vi "upload.file_multipart_upload.vi"(8 "error in":errorcluster, 10 "File Path":path, 11 "Nominal Client in":refnum<class "Nominal Client.lvclass">) -> (0 "error out":errorcluster, 2 "S3 Path to File":string, 3 "Nominal Client out":refnum<class "Nominal Client.lvclass">)   [LabVIEW 2020, in "Nominal Client.lvclass"]
doc: "Handles the upload of files in a multipart format."
uses:
  Nominal Client.lvclass
  Nominal Client MultiPart Upload/Multipart Upload.lvclass
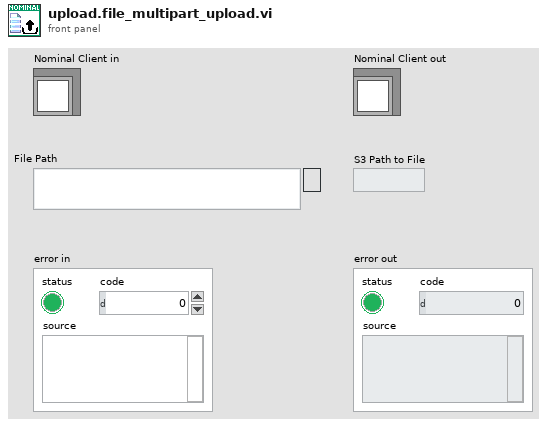
[diagram p1: front panel]
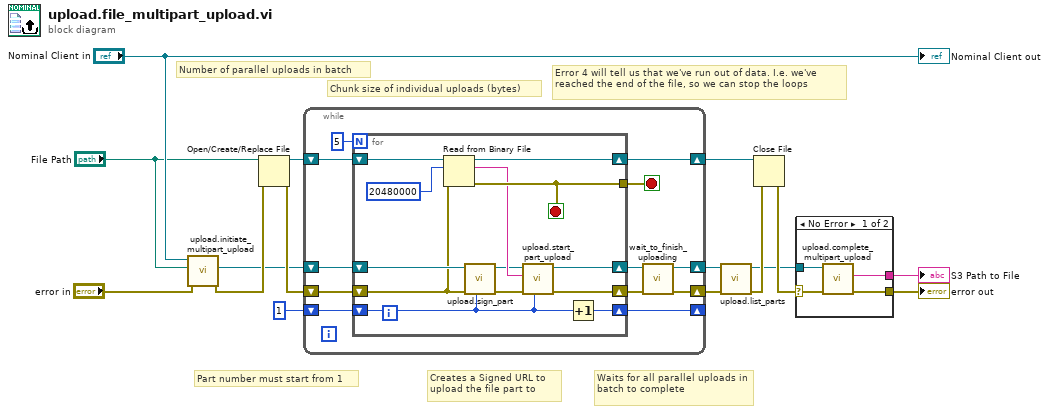
[diagram p0: block diagram]
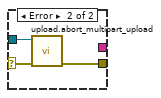
[diagram p2: hidden frame]
diagram:
  # "Waits for all parallel uploads in batch to complete"
  # "Creates a Signed URL to upload the file part to"
  # "Chunk size of individual uploads (bytes)"
  # "Number of parallel uploads in batch"
  # "Part number must start from 1"
  # "Error 4 will tell us that we've run out of data. I.e. we've reached the end of the file, so we can stop the loops"
  n1 = call "upload.initiate_multipart_upload.vi"("error in"="error in", "File Path"="File Path", "Nominal Client in"="Nominal Client in") -> ("error out"=w11:errorcluster, "Multipart Upload"=w9:refnum<class "Multipart Upload.lvclass">)  [unwired: 6 in, 1 out]
  n2 = Open/Create/Replace File(file path (use dialog)="File Path", error in=w11) -> (refnum out=w14:refnum<file>, error out=w10:errorcluster)  [unwired: 4 in, 1 out]
  n3 = while {
    shift-right: [w17] -> w16
    shift-left: w9 -> [w28]
    shift-right: [w20] -> w12
    shift-left: w10 -> [w22]
    shift-right: [w26] -> _
    shift-left: 1 -> [w27]
    shift-right: [w23] -> w13
    shift-left: w14 -> [w25]
    stop <- w24 stop-if-true
    n4 = for {
      N: 5 -> [_]
      shift-right: [w31] -> w18
      shift-left: w28 -> [w41]
      shift-right: [w40] -> w26
      shift-left: w27 -> [w30]
      tunnel: [w36] -> w24
      shift-right: [w37] -> w23
      shift-left: w25 -> [w38]
      shift-right: [w34] -> w21
      shift-left: w22 -> [w29]
      stop <- w36 stop-if-true
      n5 = Read from Binary File(8:w29, 10:20480000 ("count (1)"), 11:w38) -> (0:w36:errorcluster, 2:w33:string, 3:w37:refnum<file>)  [unwired: 3 in, 1 out]
      n6 = call "upload.sign_part.vi"("Part Number"=w30, "error in"=w29, "Multipart Upload in"=w41) -> ("error out"=w35:errorcluster, "Multipart Upload out"=w32:refnum<class "Multipart Upload.lvclass">)  [unwired: 7 in]
      n7 = call "upload.start_part_upload.vi"("Part Number"=w30, "error in"=w35, "File Part Binary"=w33, "Multipart Upload"=w32) -> ("error out"=w34:errorcluster, "Multipart Upload out"=w31:refnum<class "Multipart Upload.lvclass">)  [unwired: 6 in]
      n8 = Increment(x=w30) -> (x+1=w40:i32)
    }
    n9 = call "wait_to_finish_uploading.vi"("error in"=w21, "Multipart Upload in"=w18) -> ("error out"=w20:errorcluster, "Multipart Upload out"=w17:refnum<class "Multipart Upload.lvclass">)  [unwired: 8 in]
  }
  n10 = call "upload.list_parts.vi"("error in"=w12, "Multipart Upload"=w16) -> ("error out"=w8:errorcluster, "Multipart Upload out"=w6:refnum<class "Multipart Upload.lvclass">)  [unwired: 8 in]
  n11 = Close File(refnum=w13, error in=w8) -> (error out=w7:errorcluster)  [unwired: 1 out]
  n12 = case shown="No Error" w7 {
    selector: w7 -> [w43 w48]
    tunnel: [w45 _] -> w5
    tunnel: w6 -> [w44 w47]
    tunnel: [w42 w46] -> w4
    frame No Error {
      n13 = call "upload.complete_multipart_upload.vi"("error in"=w43, "Multipart Upload in"=w44) -> ("error out"=w42:errorcluster, "S3 Path to File"=w45:string)  [unwired: 8 in]
    }
    frame Error {
      n14 = call "upload.abort_multipart_upload.vi"("error in"=w48, "Multipart Upload"=w47) -> ("error out"=w46:errorcluster)  [unwired: 9 in]
    }
  }
  "error out" <- w4
  "S3 Path to File" <- w5
  "Nominal Client out" <- "Nominal Client in"
